vi "Variable glob alertes ecart temperatures.vi"() -> ()   [LabVIEW 2022 SP3]
panel:
  out "Groupe ON":bool[](array[boolean])
  out "Liste ecart temp":string[](array[string])
  in  "groupes ecart temp":T1(array[cluster])
  in  "Al temp ecart en cours":bool
  # "Alertes écart températures"
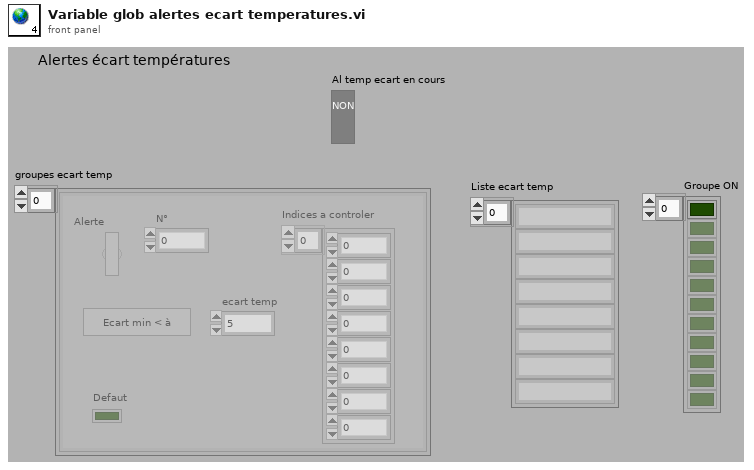
[diagram p1: front panel]
types:
  T1 = cluster{"Indices a controler":i16[], "Defaut":bool, "ecart temp":dbl, "Alerte":bool, ">?":bool, "N°":u16}[]
diagram:
